vi "Change Control Reference.vi"(8 "error in":errorcluster, 10 "Ctl Refnum":refnum<vi>, 11 "BigMAQ in":refnum<class "BigMAQ.lvclass">) -> (0 "error out":errorcluster, 1 "Image Control":T1, 3 "BigMAQ out":refnum<class "BigMAQ.lvclass">)   [LabVIEW 2019, in "BigMAQ.lvclass"]
uses:
  BigMAQ.lvclass
  <vilib>/vision/Image Controls.llb/IMAQ Image.ctl
  BigMAQ.lvclass/BigMAQ.ctl
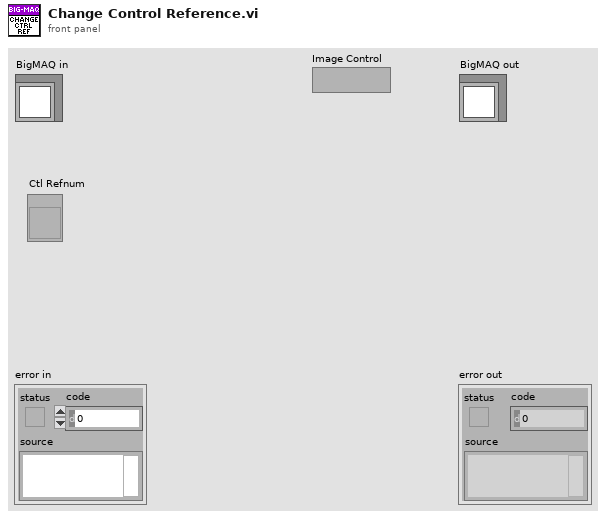
[diagram p1: front panel]
types:
  T1 = typedef "IMAQ Image.ctl" = refnum<image>
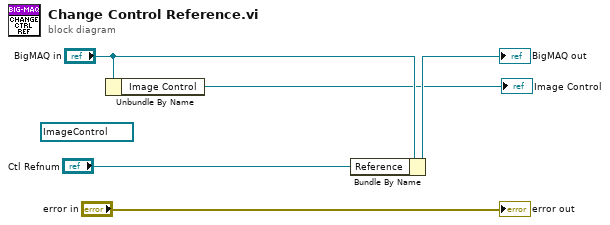
[diagram p0: block diagram]
diagram:
  (unwired) refnum<vi> refnum ("reference")
  n1 = Unbundle By Name("BigMAQ in") -> ("Image Control"=→"Image Control":T1)
  n2 = Bundle By Name(cluster="BigMAQ in", "Reference"="Ctl Refnum") -> (→"BigMAQ out":refnum<class "BigMAQ.lvclass">)
  "error out" <- "error in"
